vi "AIT 664 Main Page.vi"(8 "error in (no error)":errorcluster, 11 "Node Ptr":T1 format="%.0x") -> (0 "error out":errorcluster)   [LabVIEW 2015, in "AIT 664 Custom Device.lvlib"]
uses:
  AIT 664 Custom Device.lvlib
  <vilib>/NI Veristand/Custom Device API/Custom Device Item Ref.ctl
  Controls and Global/Global.vi
  <vilib>/NI Veristand/Custom Device API/Get Item Property (Path).vi
  <vilib>/NI Veristand/Custom Device API/Get Item Property (String).vi
  <vilib>/NI Veristand/Custom Device API/Get Item Property (Boolean).vi
  <vilib>/NI Veristand/Custom Device API/Set Item Property (String).vi
  <vilib>/NI Veristand/Custom Device API/Set Item Property (Boolean).vi
  <vilib>/NI Veristand/Custom Device API/Custom Device API.lvlib
panel:
  in  "Force Regenerate Hex File":bool
  in  "VISA Resource Address":string
  out "Database File":path
  out "MAC Address":string
  out "Network Speed":string
  out "Version":string
  in  "Header":cluster{"Section Name":string}={"Section Name"="AIT 664 Device"}
  in  "Description":string
  out "Name":string
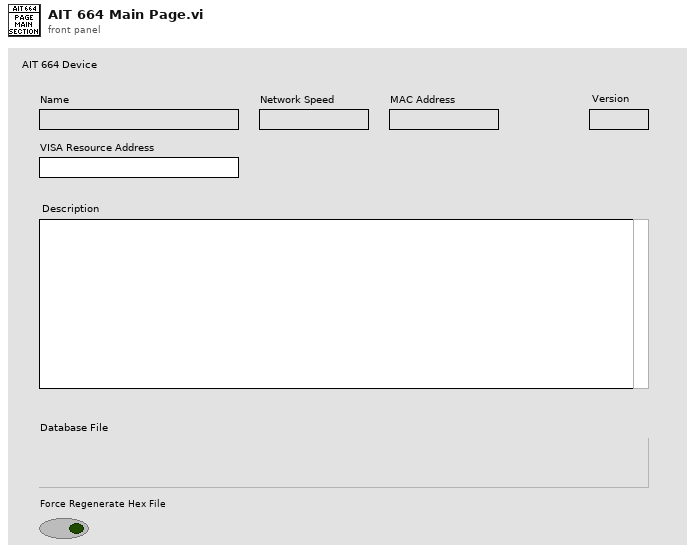
[diagram p1: front panel]
types:
  T1 = typedef "Custom Device API.lvlib/Custom Device Item Ref.ctl" = u64
  T2 = typedef "Custom Device API.lvlib/Custom Device Item Info.ctl" = cluster{"Name":string, "Is Channel":bool, "GUID":string, "Is Waveform":bool}
  T3 = typedef "Custom Device API.lvlib/Custom Device Commands.ctl" = enum16{"Default", "Item renamed", "Shutdown", "Dynamic button pressed"}
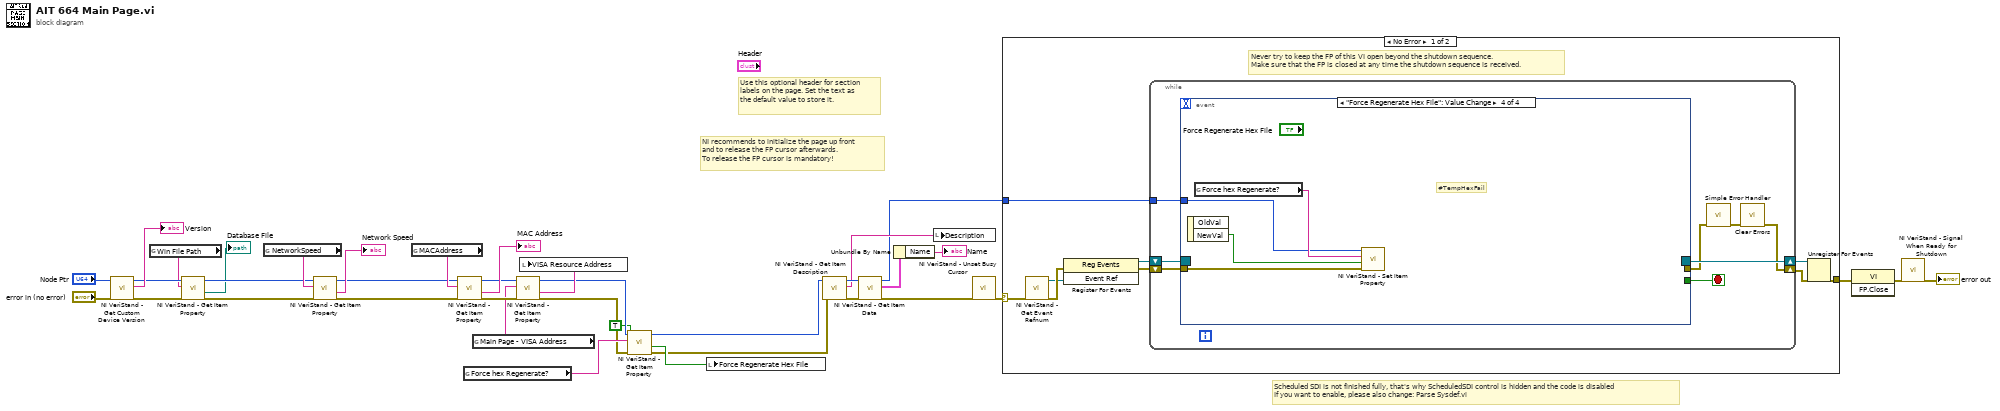
[diagram p0: block diagram]
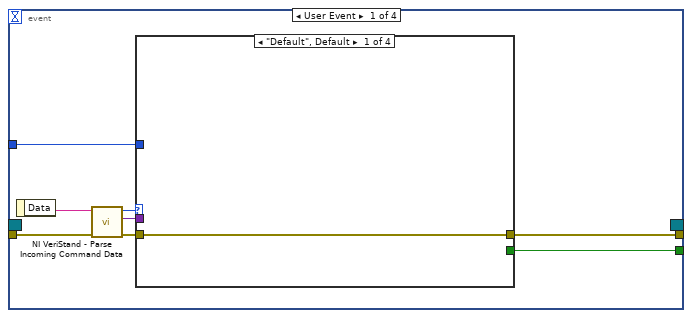
[diagram p2: hidden frame]
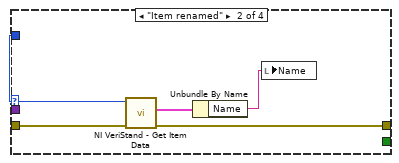
[diagram p3: hidden frame]
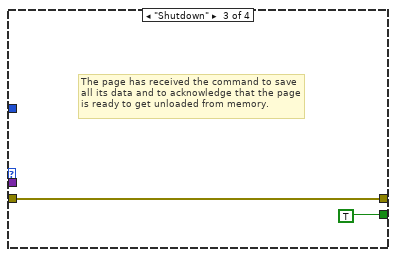
[diagram p4: hidden frame]
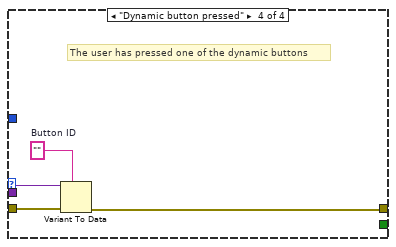
[diagram p5: hidden frame]
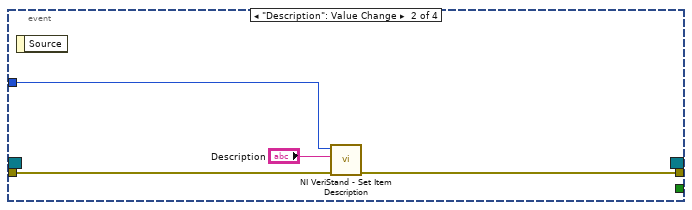
[diagram p6: hidden frame]
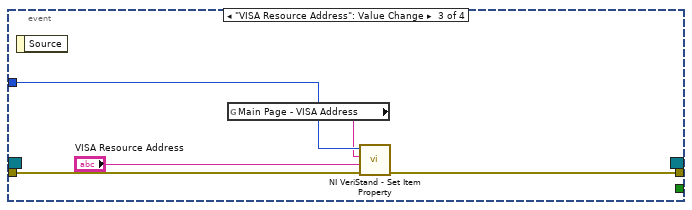
[diagram p7: hidden frame]
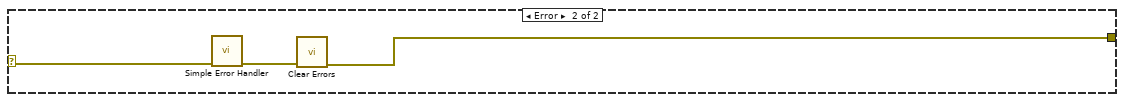
[diagram p8: hidden frame]
diagram:
  # "Scheduled SDI is not finished fully, that's why ScheduledSDI control is hidden and the code is disabled\nIf you want to enable, please also change: Parse Sysdef.vi"
  # "Use this optional header for section labels on the page. Set the text as the default value to store it."
  # "NI recommends to initialize the page up front\nand to release the FP cursor afterwards.\nTo release the FP cursor is mandatory!"
  n1 = call <vilib>:"NI VeriStand - Get Custom Device Version.vi"("error in (no error)"="error in (no error)", "Device Ref in"="Node Ptr") -> ("error out"=w17:errorcluster, "Value"=→"Version":string, "Device Ref out"=w15:T1)  [unwired: 7 in]
  n2 = global read "Global.vi" "Win File Path"() -> (w13:string)
  n3 = call-poly <vilib>:"NI VeriStand - Get Item Property.vi"("error in (no error)"=w17, "Property Name"=w13, "Item Ref in"=w15) -> ("error out"=w16:errorcluster, "Value"=→"Database File":path, "Item Ref out"=w14:T1)  [unwired: 5 in, 1 out]
  n4 = global read "Global.vi" "NetworkSpeed"() -> (w24:string)
  n5 = call-poly <vilib>:"NI VeriStand - Get Item Property.vi"("error in (no error)"=w16, "Property Name"=w24, "Item Ref in"=w14) -> ("error out"=w19:errorcluster, "Value"=→"Network Speed":string, "Item Ref out"=w20:T1)  [unwired: 5 in, 1 out]
  n6 = global read "Global.vi" "MACAddress"() -> (w21:string)
  n7 = call-poly <vilib>:"NI VeriStand - Get Item Property.vi"("error in (no error)"=w19, "Property Name"=w21, "Item Ref in"=w20) -> ("error out"=w10:errorcluster, "Value"=→"MAC Address":string, "Item Ref out"=w11:T1)  [unwired: 5 in, 1 out]
  n8 = global read "Global.vi" "Force hex Regenerate?"() -> (w5:string)
  n9 = global read "Global.vi" "Main Page - VISA Address"() -> (w9:string)
  n10 = call-poly <vilib>:"NI VeriStand - Get Item Property.vi"("error in (no error)"=w10, "Property Name"=w9, "Item Ref in"=w11) -> ("error out"=w4:errorcluster, "Value"=w8:string, "Item Ref out"=w7:T1)  [unwired: 5 in, 1 out]
  n11 = local write "VISA Resource Address"(w8) -> ()
  n12 = call-poly <vilib>:"NI VeriStand - Get Item Property.vi"("error in (no error)"=w4, "Default Value"=TRUE, "Property Name"=w5, "Item Ref in"=w7) -> ("error out"=w2:errorcluster, "Value"=w3:bool, "Item Ref out"=w6:T1)  [unwired: 4 in, 1 out]
  n13 = local write "Force Regenerate Hex File"(w3) -> ()
  n14 = call <vilib>:"NI VeriStand - Get Item Description.vi"("error in (no error)"=w2, "Item Ref in"=w6) -> ("error out"=w30:errorcluster, "Description"=w31:string, "Item Ref out"=w32:T1)  [unwired: 7 out]
  n15 = call <vilib>:"NI VeriStand - Get Item Data.vi"("error in (no error)"=w30, "Item Ref in"=w32) -> ("error out"=w34:errorcluster, "Item Info"=w29:T2, "Item Ref out"=w25:T1)  [unwired: 7 out]
  n16 = Unbundle By Name(w29) -> ("Name"=→"Name":string)
  n17 = local write "Description"(w31) -> ()
  n18 = call <vilib>:"NI VeriStand - Unset Busy Cursor.vi"("error in (no error)"=w34) -> ("error out"=w33:errorcluster)  [unwired: 10 out]
  n19 = case shown="No Error" w33 {
    selector: w33 -> [w38 w90]
    tunnel: [w43 w88] -> w37
    tunnel: w25 -> [w39 _]
    frame No Error {
      # "Never try to keep the FP of this VI open beyond the shutdown sequence.\nMake sure that the FP is closed at any time the shutdown sequence is received."
      n20 = call <vilib>:"NI VeriStand - Get Event Refnum.vi"("error in (no error)"=w38) -> ("error out"=w46:errorcluster, "Event Ref"=w42:refnum<user-event>)  [unwired: 9 out]
      n21 = register-events(error in=w46, w42) -> (reference out=w40:refnum<event-registration>, error out=w41:errorcluster)  [unwired: 1 in]
      n22 = while {
        tunnel: w39 -> [w50]
        shift-right: [w47] -> w44
        shift-left: w41 -> [w53]
        shift-right: [w54] -> w45
        shift-left: w40 -> [w52]
        stop <- w51 stop-if-true
        n23 = event shown="[3] \"Force Regenerate Hex File\": Value Change" {
          selector: w52 -> [_ _ _ _]
          dyn-events: [_ _ _ _] -> w54
          timeout: _ -> [_ _ _ _]
          tunnel: w53 -> [w62 w77 w82 w87]
          tunnel: [w58 _ _ _] -> w51
          tunnel: [w57 w76 w83 _] -> w49
          tunnel: w50 -> [w56 w78 w81 w85]
          event User Event {
            n24 = event-data() -> ("Data"=w61:string)  [unwired: 1 out]
            n25 = call <vilib>:"NI VeriStand - Parse Incoming Command Data.vi"("error in (no error)"=w62, "Incoming data"=w61) -> ("error out"=w60:errorcluster, "Outgoing data"=w55:variant, "Action"=w59:T3)  [unwired: 7 out]
            n26 = case shown="\"Default\", Default" w59 {
              tunnel: w60 -> [w63 w68 w69 w74]
              tunnel: [_ _ TRUE _] -> w58
              tunnel: [w63 w65 w69 w71] -> w57
              tunnel: w56 -> [_ w67 _ _]
              tunnel: w55 -> [_ _ _ w73]
              frame "Default", Default {
              }
              frame "Item renamed" {
                n27 = call <vilib>:"NI VeriStand - Get Item Data.vi"("error in (no error)"=w68, "Item Ref in"=w67) -> ("error out"=w65:errorcluster, "Item Info"=w66:T2)  [unwired: 8 out]
                n28 = Unbundle By Name(w66) -> ("Name"=w64:string)
                n29 = local write "Name"(w64) -> ()
              }
              frame "Shutdown" {
                # "The page has received the command to save all its data and to acknowledge that the page is ready to get unloaded from memory."
              }
              frame "Dynamic button pressed" {
                w72 = ""  # Button ID
                # "The user has pressed one of the dynamic buttons"
                n30 = Variant To Data(error in=w74, type=w72, Variant=w73) -> (error out=w71:errorcluster)  [unwired: 1 out]
              }
            }
          }
          event "Description": Value Change {
            n31 = event-data() -> ()  [unwired: 2 out]
            n32 = call <vilib>:"NI VeriStand - Set Item Description.vi"("error in (no error)"=w77, "Description"="Description", "Item Ref in"=w78) -> ("error out"=w76:errorcluster)  [unwired: 8 out]
          }
          event "VISA Resource Address": Value Change {
            n33 = event-data() -> ()  [unwired: 2 out]
            n34 = global read "Global.vi" "Main Page - VISA Address"() -> (w79:string)
            n35 = call-poly <vilib>:"NI VeriStand - Set Item Property.vi"("error in (no error)"=w82, "Value"="VISA Resource Address", "Property Name"=w79, "Item Ref in"=w81) -> ("error out"=w83:errorcluster)  [unwired: 5 in, 2 out]
          }
          event "Force Regenerate Hex File": Value Change {
            # "#TempHexFail"
            n36 = event-data() -> ("NewVal"=w84:bool)  [unwired: 2 out]
            n37 = global read "Global.vi" "Force hex Regenerate?"() -> (w86:string)
            n38 = call-poly <vilib>:"NI VeriStand - Set Item Property.vi"("error in (no error)"=w87, "Value"=w84, "Property Name"=w86, "Item Ref in"=w85) -> ()  [unwired: 5 in, 3 out]
          }
        }
        n39 = call <vilib>:"Simple Error Handler.vi"("error in (no error)"=w49) -> ("error out"=w48:errorcluster)  [unwired: 1 in, 7 out]
        n40 = call <vilib>:"Clear Errors.vi"("error in (no error)"=w48) -> ("error out"=w47:errorcluster)  [unwired: 1 in, 5 out]
      }
      n41 = Unregister For Events(event registration refnum=w45, error in=w44) -> (error out=w43:errorcluster)
    }
    frame Error {
      n42 = call <vilib>:"Simple Error Handler.vi"("error in (no error)"=w90) -> ("error out"=w89:errorcluster)  [unwired: 1 in, 7 out]
      n43 = call <vilib>:"Clear Errors.vi"("error in (no error)"=w89) -> ("error out"=w88:errorcluster)  [unwired: 1 in, 5 out]
    }
  }
  n44 = invoke class="VI" method="FP.Close"(error in=w37) -> (error out=w36:errorcluster)  [unwired: 2 in, 2 out]
  n45 = call <vilib>:"NI VeriStand - Signal When Ready for Shutdown.vi"("error in (no error)"=w36) -> ("error out"=→"error out":errorcluster)  [unwired: 10 out]
